vi "Actor Core.vi"(8 "error in":errorcluster caption="错误输入", 11 "VoiceControl in":refnum<class "Voice.lvclass"> caption="操作者输入") -> (0 "error out":errorcluster caption="错误输出", 3 "Actor out":refnum<class "Actor.lvclass"> caption="操作者输出")   [LabVIEW 2014, in "Voice.lvlib" / "Voice.lvclass"]
doc: "(<B>文件名</B>：Actor Framework.lvlib:Actor.lvclass:Actor Core.vi)\n\n接收发送至操作者的消息，响应消息并处理可能导致操作者关闭的错误。\n\n子孙类重写该VI，使操作者完成特定的任务。使用调用父方法节点实现重写。"
uses:
  Voice.lvclass
  <vilib>/ActorFramework/Actor/Actor.lvclass
  <vilib>/ActorFramework/Actor/Actor.lvclass/Actor.ctl
  Voice.lvclass/Voice.ctl
  <vilib>/ActorFramework/Message Enqueuer/Message Enqueuer.lvclass/Message Enqueuer.ctl
  <vilib>/ActorFramework/Message Enqueuer/Enqueue.vi
  <vilib>/ActorFramework/Message Priority Queue/Priority Enqueue.vi
  <vilib>/regexp/Match Regular Expression.xnode
panel:
  out "standard error":string caption="命令行执行错误"
  out "error out 2":errorcluster caption="Python执行错误"
  out "格式化机器人指令":string[][](array[string])
  out "语音信号输出字符串":string
  in  "停止信号":bool
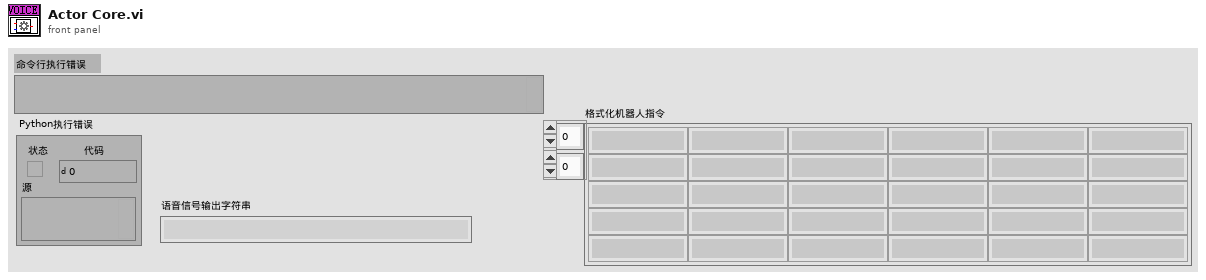
[diagram p1: front panel]
types:
  T1 = cluster{"Stop":refnum<user-event>, "Text":refnum<user-event>, "Connected":refnum<user-event>}
  T2 = enum16{"Standard", "Buffered", "CRLF", "Immediate"}
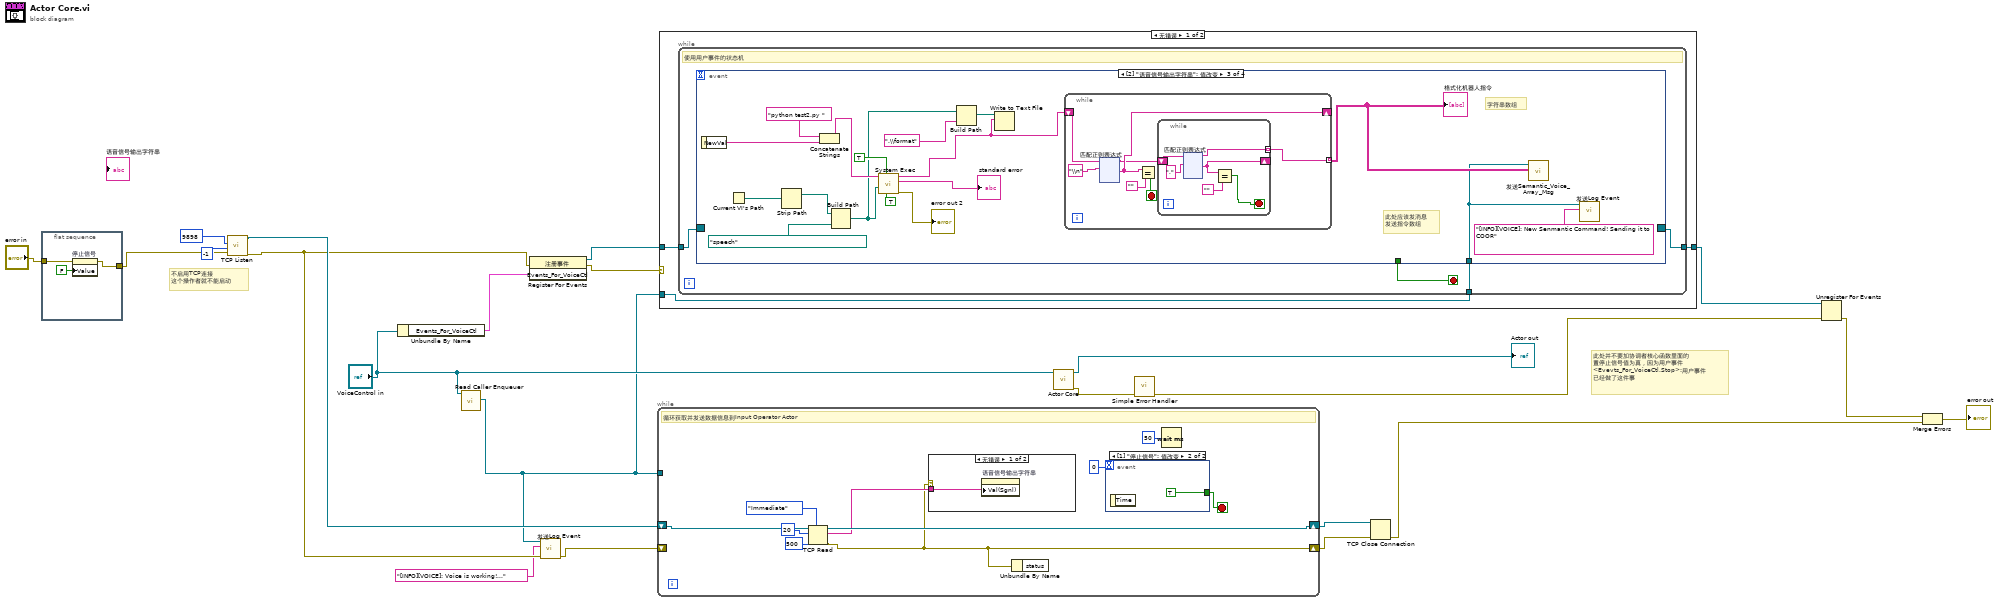
[diagram p0: block diagram]
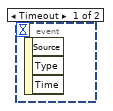
[diagram p3: hidden frame]
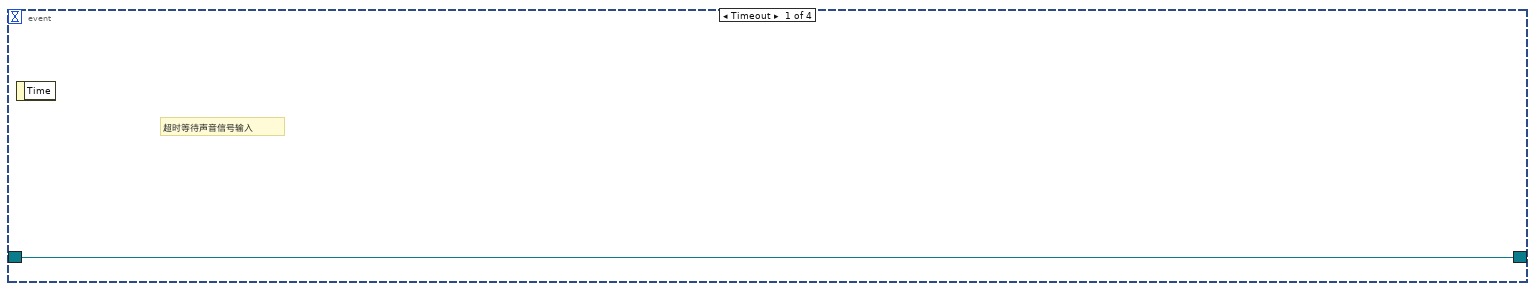
[diagram p4: hidden frame]
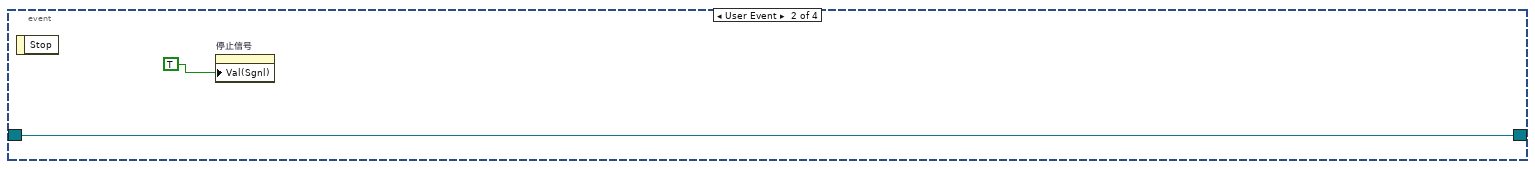
[diagram p5: hidden frame]
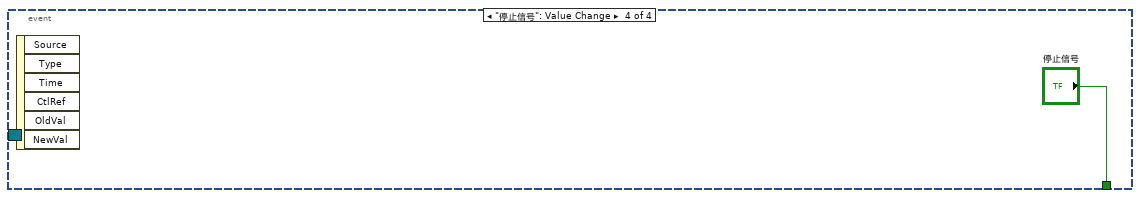
[diagram p6: hidden frame]
diagram:
  # "不启用TCP连接\n这个操作者就不能启动"
  # "此处并不要加协调者核心函数里面的\n置停止信号值为真，因为用户事件\n<Evevts_For_VoiceCtl.Stop>:用户事件\n已经做了这件事"
  n1 = flat-sequence {
    tunnel: "error in" -> [w25]
    tunnel: [w23] -> w5
    frame #0 {
      n2 = property on="停止信号" class="Bool (严格)"(error in=w25, "Value"=FALSE ("停止信号")) -> (error out=w23:errorcluster)  [unwired: 1 in, 1 out]
    }
  }
  n3 = call <vilib>:"TCP Listen.vi"("error in (no error)"=w5, "timeout ms (wait forever: -1)"=-1, "port"=u16 9898) -> ("error out"=w4:errorcluster, "connection ID"=w9:refnum<k5>)  [unwired: 4 in, 3 out]
  n4 = Unbundle By Name("VoiceControl in") -> ("Events_For_VoiceCtl"=w21:T1)
  n5 = call <vilib>:"Read Caller Enqueuer.vi"("Actor"="VoiceControl in") -> ("Caller Enqueuer"=w2:refnum<class "Message Enqueuer.lvclass">)  [unwired: 10 in]
  n6 = register-events(error in=w4, w21) -> (reference out=w20:refnum<event-registration>, error out=w18:errorcluster)  [unwired: 1 in]
  n7 = call "发送Log Event.vi"("error in (no error)"=w4, "Event Text"="[INFO][VOICE]: Voice is working!...", "消息待入队列"=w2) -> ("error out"=w3:cluster{"状态":bool, "代码":i32, "源":string})  [unwired: 7 in, 1 out]
  n8 = while {
    tunnel: w2 -> [_]
    shift-right: [w32] -> w7
    shift-left: w9 -> [w29]
    shift-right: [w30] -> w6
    shift-left: w3 -> [_]
    stop <- w33 stop-if-true
    # "循环获取并发送数据信息到Input Operator Actor"
    n9 = TCP Read(connection ID=w29, bytes to read=20 ("读取的字节"), 7:T2."Immediate" ("模式（标准）"), 9:500 ("超时毫秒(25000)")) -> (connection ID out=w32:refnum<k5>, data out=w31:string, error out=w30:errorcluster)  [unwired: 1 in]
    n10 = case shown="无错误" w30 {
      tunnel: w31 -> [w36 _]
      frame No Error {
        n11 = property on="语音信号输出字符串" class="Str"("Val(Sgnl)"=w36) -> ()  [unwired: 2 in, 2 out]
      }
      frame Error {
      }
    }
    n12 = Unbundle By Name(w30) -> ()  [unwired: 1 out]
    n13 = event shown="[1] \"停止信号\": 值改变" {
      selector: _ -> [_ _]
      dyn-events: _ -> [_ _]
      timeout: 0 -> [_ _]
      tunnel: [_ TRUE] -> w33
      event Timeout {
        n14 = event-data() -> ()  [unwired: 1 in, 3 out]
      }
      event "停止信号": Value Change {
        n15 = event-data() -> ()  [unwired: 1 in, 1 out]
      }
    }
    n16 = Wait (ms)(milliseconds to wait=u32 50 ("等待时间（毫秒）")) -> ()  [unwired: 1 out]
  }
  n17 = case shown="无错误" w18 {
    tunnel: [w40 w307] -> w14
    tunnel: w20 -> [w39 w307]
    tunnel: w2 -> [w38 _]
    frame No Error {
      n18 = while {
        tunnel: [w43] -> w40
        tunnel: w39 -> [w42]
        tunnel: w38 -> [w41]
        stop <- w44 stop-if-true
        # "使用用户事件的状态机"
        n19 = event shown="[2] \"语音信号输出字符串\": 值改变" {
          selector: w42 -> [w45 w47 _ _]
          dyn-events: [w45 w47 _ _] -> w43
          timeout: _ -> [_ _ _ _]
          tunnel: [_ _ _ "停止信号"] -> w44
          tunnel: w41 -> [_ _ w50 _]
          event Timeout {
            # "超时等待声音信号输入"
            n20 = event-data() -> ()  [unwired: 1 in, 1 out]
          }
          event User Event {
            n21 = event-data() -> ()  [unwired: 1 in, 1 out]
            n22 = property on="停止信号" class="Bool (严格)"("Val(Sgnl)"=TRUE) -> ()  [unwired: 2 in, 2 out]
          }
          event "语音信号输出字符串": Value Change {
            # "字符串数组"
            # "此处应该发消息\n发送指令数组"
            n23 = event-data() -> ("NewVal"=w56:string)  [unwired: 1 in]
            n24 = Current VI's Path() -> (path=w52:path)
            n25 = Strip Path(path=w52) -> (stripped path=w54:path)  [unwired: 1 out]
            n26 = Concatenate Strings("python test2.py " ("command line"), w56) -> (w61:string)
            n27 = Build Path(base path=w54, name or relative path=path "speech") -> (appended path=w53:path)
            n28 = call <vilib>:"System Exec.vi"("run minimized? (F)"=TRUE, "wait until completion? (T)"=TRUE, "working directory"=w53, "command line"=w61) -> ("error out"=→"error out 2":errorcluster, "standard error"=→"standard error":string, "standard output"=w64:string)  [unwired: 4 in, 1 out]
            n29 = Build Path(base path=w53, name or relative path=".\\format" ("名称或相对路径")) -> (appended path=w63:path)
            n30 = Write to Text File(file (use dialog)=w63, text=w64) -> ()  [unwired: 2 in, 3 out]
            n31 = while {
              tunnel: [w65] -> w51 mode=indexing
              shift-right: [w69] -> _
              shift-left: w64 -> [w70]
              stop <- w67 stop-if-true
              n32 = xnode "匹配正则表达式"("输入字符串"=w70, "正则表达式"="\\n") -> ("匹配之前"=w66:string, "匹配之后"=w69:string)  [unwired: 4 in, 3 out]
              n33 = Equal?(x=w69, y="") -> (x = y?=w67:bool)
              n34 = while {
                shift-right: [w73] -> _
                shift-left: w66 -> [w77]
                tunnel: [w75] -> w65 mode=indexing
                stop <- w72 stop-if-true
                n35 = xnode "匹配正则表达式"("输入字符串"=w77, "正则表达式"=",") -> ("匹配之前"=w75:string, "匹配之后"=w73:string)  [unwired: 4 in, 3 out]
                n36 = Equal?(x=w73, y="") -> (x = y?=w72:bool)
              }
            }
            "格式化机器人指令" <- w51
            n37 = call "发送Semantic_Voice_Array_Msg.vi"("Semantic_Voice_Array"=w51, "消息待入队列"=w50) -> ()  [unwired: 8 in, 2 out]
            n38 = call "发送Log Event.vi"("Event Text"="[INFO][VOICE]: New Senmantic Command! Sending it to COOR", "消息待入队列"=w50) -> ()  [unwired: 8 in, 2 out]
          }
          event "停止信号": Value Change {
            n39 = event-data() -> ()  [unwired: 1 in, 6 out]
          }
        }
      }
    }
    frame Error {
    }
  }
  n40 = call-parent "Actor Core.vi"("Actor in"="VoiceControl in") -> ("error out"=w16:errorcluster, "Actor out"=→"Actor out":refnum<class "Actor.lvclass">)  [unwired: 9 in]
  n41 = call <vilib>:"Simple Error Handler.vi"("error in (no error)"=w16) -> ("error out"=w15:errorcluster)  [unwired: 4 in, 4 out]
  n42 = TCP Close Connection(connection ID=w7, error in (no error)=w6) -> (error out=w8:errorcluster)  [unwired: 1 in, 1 out]
  n43 = Unregister For Events(event registration refnum=w14, error in=w15) -> (error out=w12:errorcluster)
  n44 = Merge Errors(w12, w8) -> (→"error out":errorcluster)
